vi "Refresh Device Info.vi"(8 "error in (no error)":errorcluster, 11 "Device in":refnum<class "Device.lvclass">) -> (0 "error out":errorcluster, 3 "Device out":refnum<class "Device.lvclass">)   [LabVIEW 2020, in "PicoG-App.lvlib" / "Device.lvclass"]
uses:
  Device.lvclass
  Device.lvclass/Device.ctl
  Builds/picoG/ppl/PicoG-Core.lvlibp/PicoG-Processor/PicoG-Core/Resource/Resource.lvclass
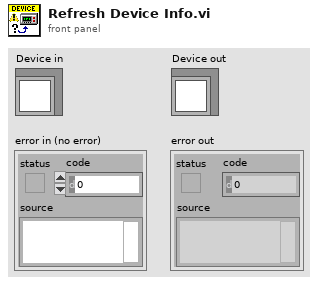
[diagram p1: front panel]
types:
  T1 = typedef "PicoG-App.lvlib/Device.lvclass/Ref Data.ctl" = cluster{"Alias":string, "Version":string, "Build":timestamp, "Key":T2}
  T2 = typedef "PicoG-App.lvlib/Device.lvclass/Device Key.ctl" = cluster{"Platform":string, "Board":string, "ID":string}
  T3 = typedef "PicoG-App.lvlib/Device.lvclass/Resource Ref.ctl" = cluster{"Resource":refnum<class "Resource.lvclass">, "Open":bool, "At Prompt":bool, "Running":bool}
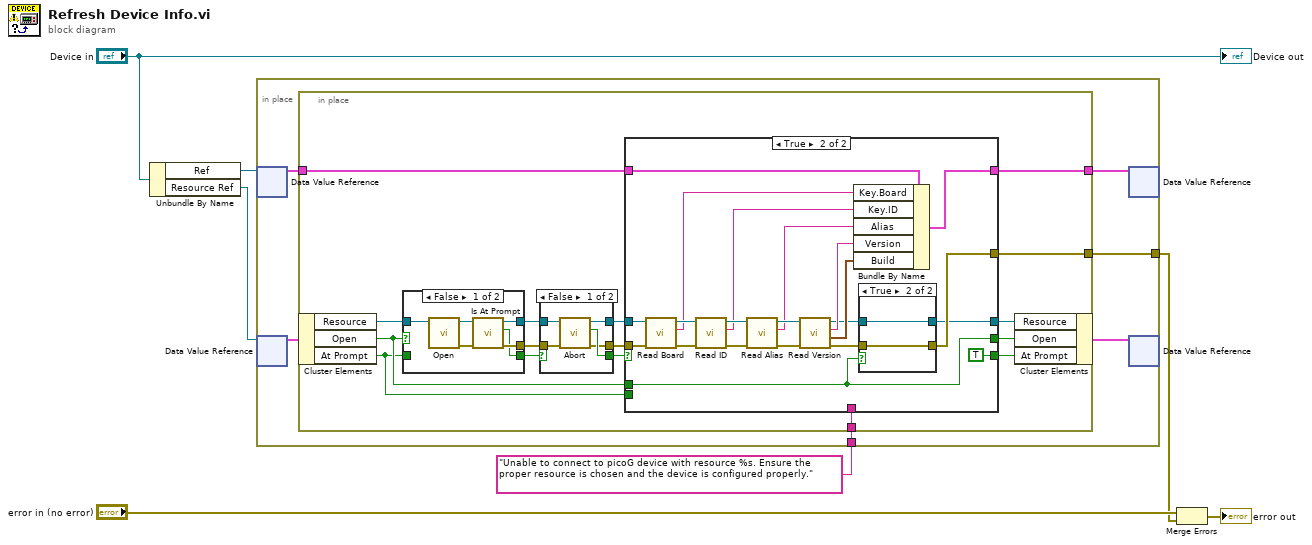
[diagram p0: block diagram]
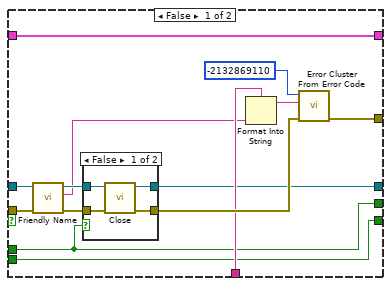
[diagram p2: hidden frame]
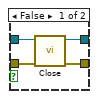
[diagram p4: hidden frame]
diagram:
  n1 = Unbundle By Name("Device in") -> ("Ref"=w6:refnum<data-value>, "Resource Ref"=w4:refnum<data-value>)
  n2 = in-place {
    in-place-border: [w11] -> w2
    in-place-border: "Unable to connect to picoG device with resource %s. Ensure the proper resource is chosen and the device is configured properly." -> [w10]
    n3 = in-place-dvr #1(w6) -> (w13:T1)  [unwired: 1 out]
    n4 = in-place-dvr #2(w4) -> (w9:T3)  [unwired: 1 out]
    n5 = in-place {
      in-place-border: w13 -> [w23]
      in-place-border: [w22] -> w12
      in-place-border: [w21] -> w11
      in-place-border: w10 -> [w20]
      n6 = in-place-cluster #3(w9) -> ("Resource"=w19:refnum<class "Resource.lvclass">, "Open"=w17:bool, "At Prompt"=w15:bool)
      n7 = case shown="False" w17 {
        tunnel: [w89 w91] -> w27
        tunnel: [w87 _] -> w28
        tunnel: [w86 w92] -> w29
        tunnel: w15 -> [_ w92]
        tunnel: w19 -> [w85 w91]
        frame False {
          n8 = call-dynamic "Open.vi"("DeployResource in"=w85) -> ("error out"=w88:errorcluster, "DeployResource out"=w90:refnum<class "Resource.lvclass">)  [unwired: 9 in]
          n9 = call-dynamic "Is At Prompt.vi"("error in (no error)"=w88, "DeployResource in"=w90) -> ("error out"=w87:errorcluster, "At Prompt?"=w86:bool, "DeployResource out"=w89:refnum<class "Resource.lvclass">)  [unwired: 6 in, 1 out]
        }
        frame True {
        }
      }
      n10 = case shown="False" w29 {
        selector: w29 -> [_ w84]
        tunnel: w28 -> [w80 w82]
        tunnel: w27 -> [w81 w83]
        tunnel: [w79 w84] -> w26
        tunnel: [w78 w82] -> w25
        tunnel: [w77 w83] -> w24
        frame False {
          n11 = call-dynamic "Abort.vi"("error in (no error)"=w80, "DeployResource in"=w81) -> ("error out"=w78:errorcluster, "Stopped?"=w79:bool, "DeployResource out"=w77:refnum<class "Resource.lvclass">)  [unwired: 6 in, 1 out]
        }
        frame True {
        }
      }
      n12 = case shown="True" w26 {
        tunnel: w25 -> [w38 w69]
        tunnel: w24 -> [w39 w70]
        tunnel: w23 -> [w42 w62]
        tunnel: [w42 w56] -> w22
        tunnel: [w40 w53] -> w21
        tunnel: w20 -> [w37 _]
        tunnel: [w32 TRUE] -> w18
        tunnel: w17 -> [w33 w51]
        tunnel: [w33 w51] -> w16
        tunnel: w15 -> [w32 _]
        tunnel: [w30 w50] -> w14
        frame False {
          n13 = call-dynamic "Friendly Name.vi"("error in (no error)"=w38, "DeployResource in"=w39) -> ("error out"=w35:errorcluster, "Friendly Name"=w31:string, "DeployResource out"=w34:refnum<class "Resource.lvclass">)  [unwired: 7 in]
          n14 = case shown="False" w33 {
            tunnel: w35 -> [w46 w48]
            tunnel: w34 -> [w47 w49]
            tunnel: [w45 w49] -> w30
            tunnel: [w44 w48] -> w43
            frame False {
              n15 = call-dynamic "Close.vi"("error in (no error)"=w46, "DeployResource in"=w47) -> ("error out"=w44:errorcluster, "DeployResource out"=w45:refnum<class "Resource.lvclass">)  [unwired: 8 in]
            }
            frame True {
            }
          }
          n16 = Format Into String(format string=w37, w31) -> (resulting string=w36:string)  [unwired: 2 in, 1 out]
          n17 = call <vilib>:"Error Cluster From Error Code.vi"("error in (no error)"=w43, "error message (\"\")"=w36, "error code (0)"=-2132869110) -> ("error out"=w40:errorcluster)  [unwired: 6 in]
        }
        frame True {
          n18 = call "Read Board.vi"("error in (no error)"=w69, "DeployResource in"=w70) -> ("error out"=w67:errorcluster, "Board"=w57:string, "DeployResource out"=w68:refnum<class "Resource.lvclass">)  [unwired: 7 in]
          n19 = call "Read ID.vi"("error in (no error)"=w67, "DeployResource in"=w68) -> ("error out"=w65:errorcluster, "ID"=w58:string, "DeployResource out"=w66:refnum<class "Resource.lvclass">)  [unwired: 7 in]
          n20 = call "Read Alias.vi"("error in (no error)"=w65, "DeployResource in"=w66) -> ("error out"=w63:errorcluster, "Alias"=w59:string, "DeployResource out"=w64:refnum<class "Resource.lvclass">)  [unwired: 7 in]
          n21 = call "Read Version.vi"("error in (no error)"=w63, "DeployResource in"=w64) -> ("error out"=w54:errorcluster, "Build"=w61:timestamp, "Version"=w60:string, "DeployResource out"=w55:refnum<class "Resource.lvclass">)  [unwired: 6 in]
          n22 = Bundle By Name(cluster=w62, "Key.Board"=w57, "Key.ID"=w58, "Alias"=w59, "Version"=w60, "Build"=w61) -> (w56:T1)
          n23 = case shown="True" w51 {
            tunnel: w55 -> [w74 w75]
            tunnel: w54 -> [w73 w76]
            tunnel: [w72 w76] -> w53
            tunnel: [w71 w75] -> w50
            frame False {
              n24 = call-dynamic "Close.vi"("error in (no error)"=w73, "DeployResource in"=w74) -> ("error out"=w72:errorcluster, "DeployResource out"=w71:refnum<class "Resource.lvclass">)  [unwired: 8 in]
            }
            frame True {
            }
          }
        }
      }
      n25 = in-place-cluster #3("Resource"=w14, "Open"=w16, "At Prompt"=w18) -> (w8:T3)
    }
    n26 = in-place-dvr #1(w12) -> ()  [unwired: 2 out]
    n27 = in-place-dvr #2(w8) -> ()  [unwired: 2 out]
  }
  n28 = Merge Errors("error in (no error)", w2) -> (→"error out":errorcluster)
  "Device out" <- "Device in"
